vi "Filter Invalid Ref.vi"(11 "Ref in":T1[](array[typedef]) format="%.0x") -> (3 "Ref out":T1[](array[typedef]) format="%.0x")   [LabVIEW 2023, in "Protection and Counter Addon System Explorer.lvlib"]
uses:
  Protection and Counter Addon System Explorer.lvlib
  <vilib>/NI VeriStand/Custom Device API/Custom Device Item Ref.ctl
  <vilib>/NI VeriStand/Custom Device API/Custom Device API.lvlib
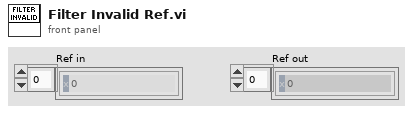
[diagram p1: front panel]
types:
  T1 = typedef "Custom Device API.lvlib/Custom Device Item Ref.ctl" = u64
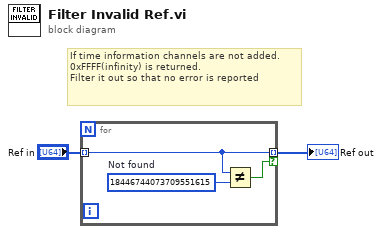
[diagram p0: block diagram]
diagram:
  # "If time information channels are not added. 0xFFFF(infinity) is returned. \nFilter it out so that no error is reported"
  n1 = for {
    tunnel: "Ref in" -> [w4] mode=indexing
    tunnel: [w4] -> w2 mode=indexing if=w3
    w5 = T1 18446744073709551615  # Not found
    n2 = Not Equal?(x=w4, y=w5) -> (x != y?=w3:bool)
  }
  "Ref out" <- w2
